vi "Sous_VI_Lanceur.vi"(11 "Nb balles":i32) -> ()   [LabVIEW 2017]
uses:
  enum_moteur_lanceur.ctl
  enum_distributeur_lanceur.ctl
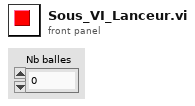
[diagram p1: front panel]
types:
  T1 = typedef "enum_moteur_lanceur.ctl" = enum16{"distance", "sans_distance", "desactive"}
  T2 = typedef "enum_distributeur_lanceur.ctl" = enum16{"Arret", "Marche"}
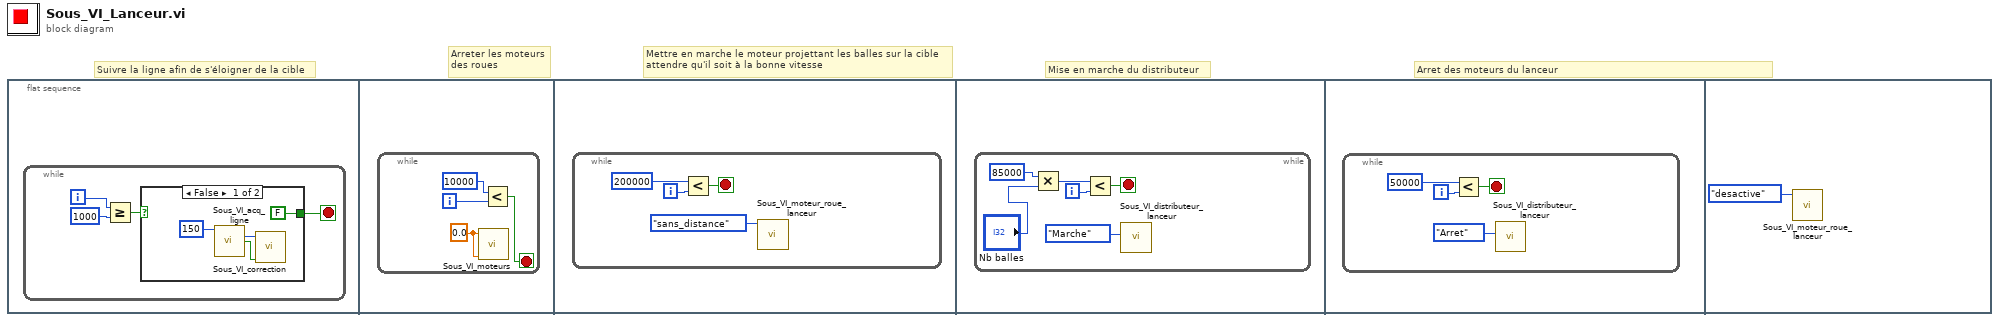
[diagram p0: block diagram]
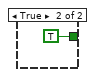
[diagram p2: hidden frame]
diagram:
  # "Arret des moteurs du lanceur"
  # "Mise en marche du distributeur"
  # "Mettre en marche le moteur projettant les balles sur la cible\nattendre qu'il soit à la bonne vitesse"
  # "Arreter les moteurs\ndes roues"
  # "Suivre la ligne afin de s'éloigner de la cible"
  n1 = flat-sequence {
    frame #0 {
      n2 = while {
        i -> [w1]
        stop <- w3 stop-if-true
        n3 = Greater Or Equal?(x=w1, y=1000) -> (x >= y?=w4:bool)
        n4 = case shown="False" w4 {
          tunnel: [FALSE TRUE] -> w3
          frame False {
            n5 = call "Sous_VI_acq_ligne.vi"("Seuil"=150) -> ("Décalage"=w7:u32, "G/D ?"=w6:bool)  [unwired: 10 in, 3 out]
            n6 = call "Sous_VI_correction.vi"("G/D ?"=w6, "Décalage"=w7) -> ()  [unwired: 10 in]
          }
          frame True {
          }
        }
      }
    }
    frame #1 {
      n7 = while {
        i -> [w12]
        stop <- w10 stop-if-true
        w13 = 0.0 ("Moteur Gauche")
        n8 = call "Sous_VI_moteurs.vi"("Moteur Droit"=w13, "Moteur Gauche"=w13) -> ()  [unwired: 10 in]
        n9 = Less?(x=10000, y=w12) -> (x < y?=w10:bool)
      }
    }
    frame #2 {
      n10 = while {
        i -> [w17]
        stop <- w15 stop-if-true
        n11 = Less?(x=200000, y=w17) -> (x < y?=w15:bool)
        n12 = call "Sous_VI_moteur_roue_lanceur.vi"("Mode"=enum_moteur_lanceur."sans_distance") -> ()  [unwired: 11 in]
      }
    }
    frame #3 {
      n13 = while {
        i -> [w23]
        stop <- w22 stop-if-true
        n14 = Multiply(x=85000, y="Nb balles") -> (x*y=w19:i32)
        n15 = Less?(x=w19, y=w23) -> (x < y?=w22:bool)
        n16 = call "Sous_VI_distributeur_lanceur.vi"("Enum"=enum_distributeur_lanceur."Marche") -> ()  [unwired: 11 in]
      }
    }
    frame #4 {
      n17 = while {
        i -> [w27]
        stop <- w25 stop-if-true
        n18 = Less?(x=50000, y=w27) -> (x < y?=w25:bool)
        n19 = call "Sous_VI_distributeur_lanceur.vi"("Enum"=enum_distributeur_lanceur."Arret") -> ()  [unwired: 11 in]
      }
    }
    frame #5 {
      n20 = call "Sous_VI_moteur_roue_lanceur.vi"("Mode"=enum_moteur_lanceur."desactive") -> ()  [unwired: 11 in]
    }
  }
